vi "Declare OpModes.vi"() -> (1 "Logging Config":T1={"Enable"=FALSE, "Log Path"=path "", "Log Flush (s)"=0.25}, 3 "OpModes":T2)   [LabVIEW 2023]
doc: "Declare the Autonomous, TeleOperated, and Utility/Test OpModes that will be displayed in the Driver Station.\nAlso defines Network Table logging configuration."
uses:
  <vilib>/MRC/MrcLib/VIs/Robot Framework/DS OpModes.ctl
panel:
  # "opModes array and logging\nconfiguration are built and\nreturned on the block diagram"
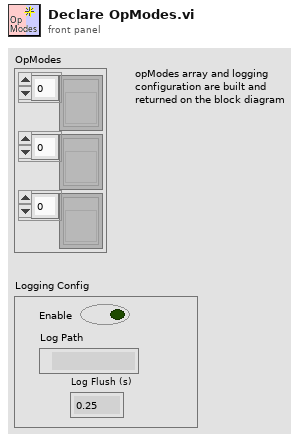
[diagram p1: front panel]
types:
  T1 = cluster{"Enable":bool, "Log Path":path, "Log Flush (s)":dbl}
  T2 = typedef "DS OpModes.ctl" = cluster{"Autos":refnum<vi>[], "Teles":refnum<vi>[], "Utilities":refnum<vi>[]}
  T3 = cluster{refnum<vi>[], refnum<vi>[], refnum<vi>[]}
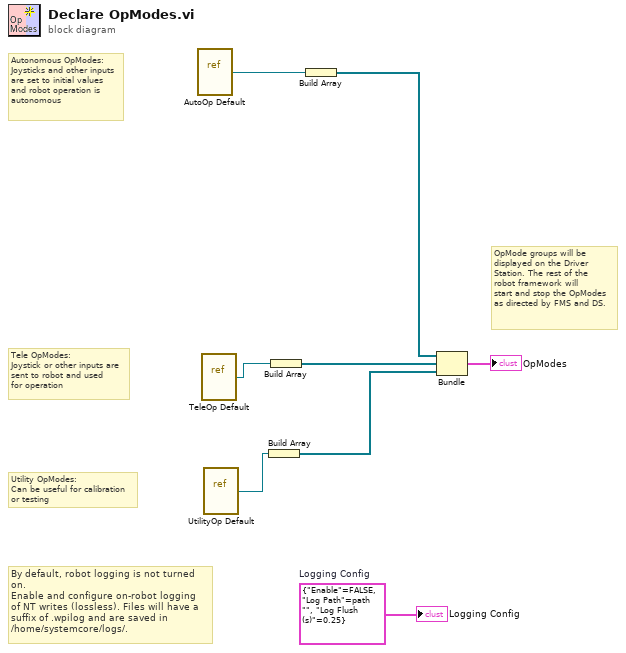
[diagram p0: block diagram]
diagram:
  w1 = T1 {"Enable"=FALSE, "Log Path"=path "", "Log Flush (s)"=0.25}  # Logging Config
  # "By default, robot logging is not turned on.\nEnable and configure on-robot logging\nof NT writes (lossless). Files will have a\nsuffix of .wpilog and are saved in \n/home/systemcore/logs/."
  # "OpMode groups will be \ndisplayed on the Driver\nStation. The rest of the \nrobot framework will\nstart and stop the OpModes\nas directed by FMS and DS."
  # "Utility OpModes:\nCan be useful for calibration\nor testing"
  # "Tele OpModes:\nJoystick or other inputs are\nsent to robot and used\nfor operation"
  # "Autonomous OpModes:\nJoysticks and other inputs\nare set to initial values\nand robot operation is\nautonomous"
  n1 = vi-ref "AutoOp Default.vi"() -> (w5:refnum<vi>)
  n2 = vi-ref "TeleOp Default.vi"() -> (w4:refnum<vi>)
  n3 = vi-ref "UtilityOp Default.vi"() -> (w3:refnum<vi>)
  n4 = Build Array(w3) -> (w7:refnum<vi>[])
  n5 = Build Array(w4) -> (w8:refnum<vi>[])
  n6 = Build Array(w5) -> (w6:refnum<vi>[])
  n7 = Bundle(w6, w8, w7) -> (→"OpModes":T3)  [unwired: 1 in]
  "Logging Config" <- w1
